vi "Every Value.vi"(8 "error in (no error)":errorcluster, 11 "prefix":string="DEV:") -> (0 "error out":errorcluster, 3 "values":map{string, refnum<class "NT Base.lvclass">}(c390))   [LabVIEW 2020]
uses:
  source/PV Data/NT Base/NT Base.lvclass
  source/PV Data/NT Scalar (Numeric)/NT Scalar (Numeric).lvclass
  C:/Users/eyw68381/source/repos/pvaccess-labview/labview/source/PV Data/NT Scalar/NT Scalar.lvclass
  C:/Users/eyw68381/source/repos/pvaccess-labview/labview/source/PV Data/NT Base/NT Base.lvclass
  source/PV Data/NT Scalar/NT Scalar.lvclass
  source/PV Data/NT Enum/NT Enum.lvclass
  source/PV Data/PV Data.lvlib
  source/PV Data/Value Fields.ctl
  source/PV Data/NT Scalar (Numeric)/Create - I64.vi
  source/PV Data/NT Scalar (Numeric)/Create - I32.vi
  source/PV Data/NT Scalar (Numeric)/Create - I16.vi
  source/PV Data/NT Scalar (Numeric)/Create - I8.vi
  source/PV Data/NT Scalar (Numeric)/Create - U16.vi
  source/PV Data/NT Scalar (Numeric)/Create - U8.vi
  source/PV Data/NT Scalar/Create - Boolean.vi
  source/PV Data/NT Scalar/Create - String.vi
  source/PV Data/NT Scalar (Numeric)/Create - DBL Array.vi
  source/PV Data/NT Scalar (Numeric)/Create - SGL Array.vi
  source/PV Data/NT Scalar (Numeric)/Create - I64 Array.vi
  source/PV Data/NT Scalar (Numeric)/Create - I32 Array.vi
  source/PV Data/NT Scalar (Numeric)/Create - I16 Array.vi
  source/PV Data/NT Scalar (Numeric)/Create - I8 Array.vi
  source/PV Data/NT Scalar (Numeric)/Create - U64 Array.vi
  source/PV Data/NT Scalar (Numeric)/Create - U32 Array.vi
  source/PV Data/NT Scalar (Numeric)/Create - U16 Array.vi
  source/PV Data/NT Scalar (Numeric)/Create - U8 Array.vi
  source/PV Data/NT Scalar/Create - Boolean Array.vi
  source/PV Data/NT Scalar/Create - String Array.vi
  source/PV Data/NT Enum/Create - Enum.vi
  source/PV Data/Display Form.ctl
  source/PV Data/NT Scalar (Numeric)/Create - SGL.vi
  source/PV Data/NT Scalar (Numeric)/Create - DBL.vi
  source/PV Data/NT Scalar (Numeric)/Create - U64.vi
  source/PV Data/NT Scalar (Numeric)/Create - U32.vi
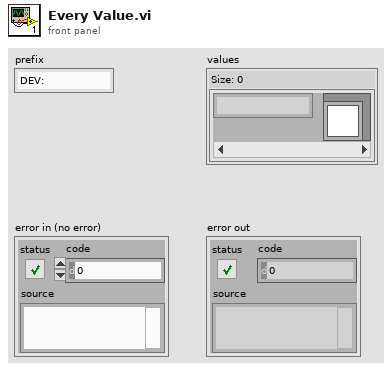
[diagram p1: front panel]
types:
  T1 = typedef "PV Access.lvlib/PV Data.lvlib/Display Form.ctl" = enum16{"Default", "String", "Binary", "Decimal", "Hex", "Exponential", "Engineering"}
  T2 = typedef "PV Access.lvlib/PV Data.lvlib/Value Fields.ctl" = cluster{"Display":bool, "Control":bool, "Alarm Limits":bool}
  T3 = typedef "PV Access.lvlib/PV Data.lvlib/Type Code.ctl" = enum8{"Null", "Bool", "BoolA", "Int8", "Int8A", "Int16", "Int16A", "Int32", "Int32A", "Int64", "Int64A", "UInt8", "UInt8A", "UInt16", "UInt16A", "UInt32", "UInt32A", "UInt64", "UInt64A", "Float32", "Float32A", "Float64", "Float64A", "String", "StringA", "Struct", "StructA", "Union", "UnionA", "Any", "AnyA"}
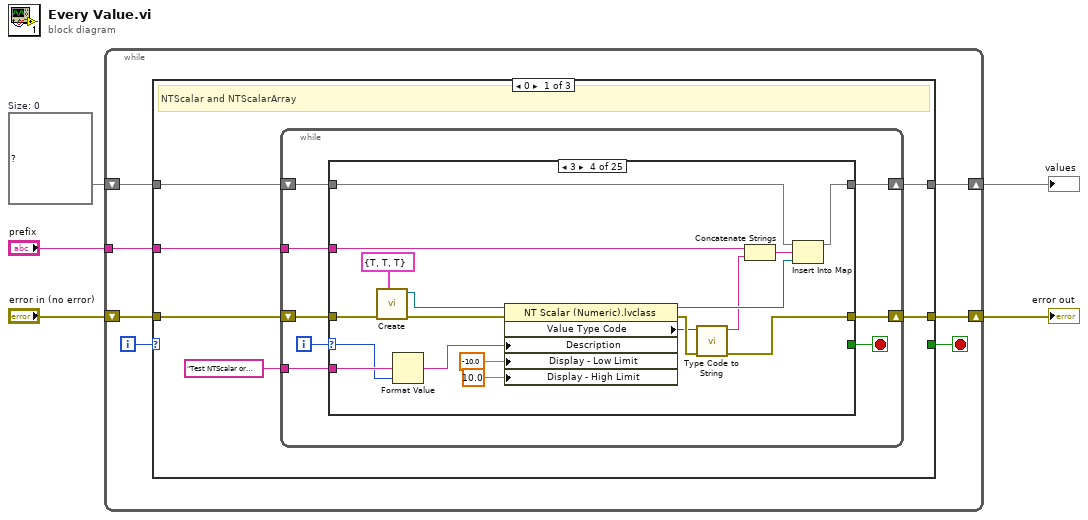
[diagram p0: block diagram]
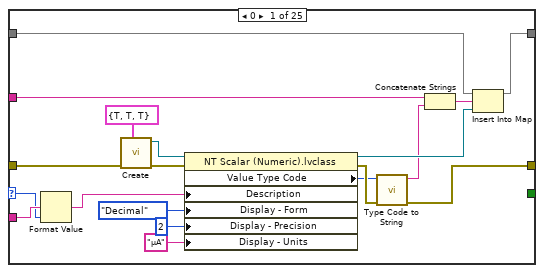
[diagram p2: hidden frame]
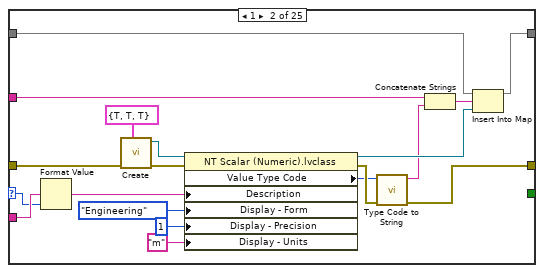
[diagram p3: hidden frame]
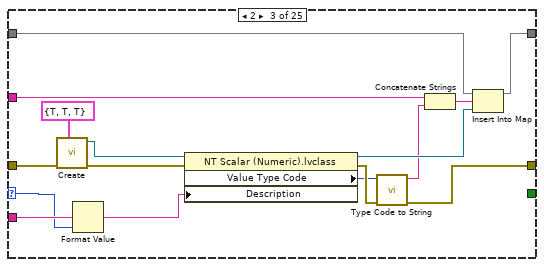
[diagram p4: hidden frame]
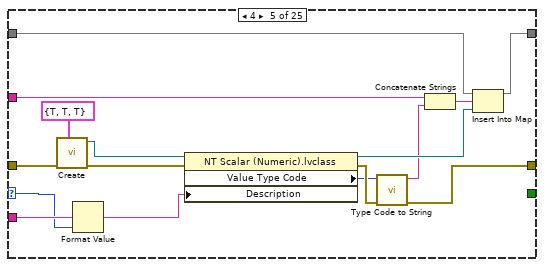
[diagram p5: hidden frame]
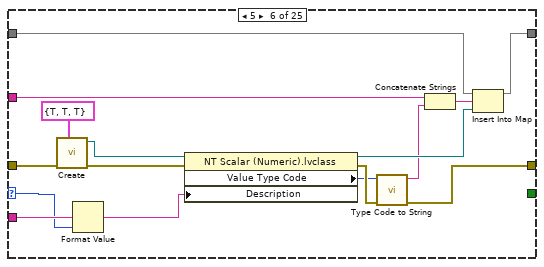
[diagram p6: hidden frame]
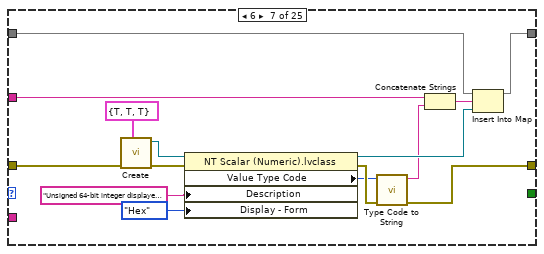
[diagram p7: hidden frame]
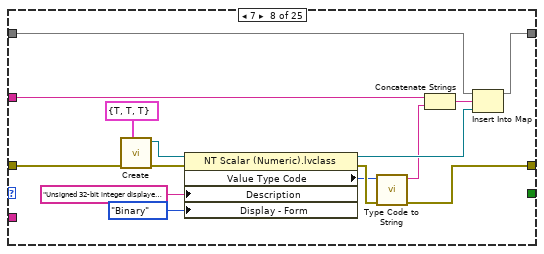
[diagram p8: hidden frame]
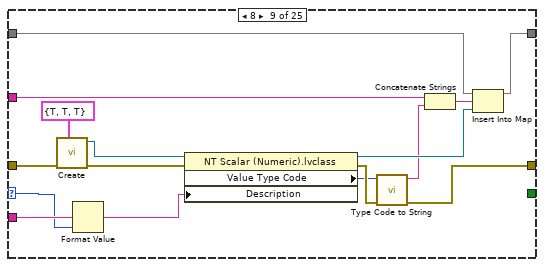
[diagram p9: hidden frame]
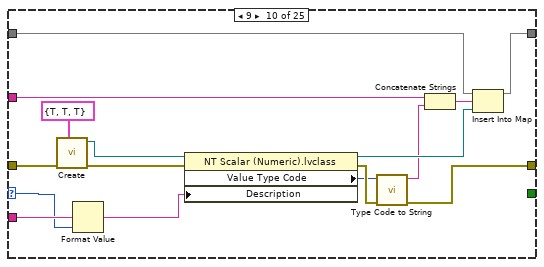
[diagram p10: hidden frame]
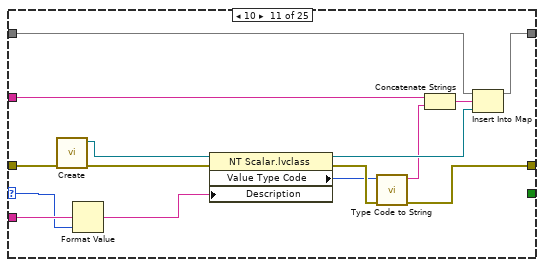
[diagram p11: hidden frame]
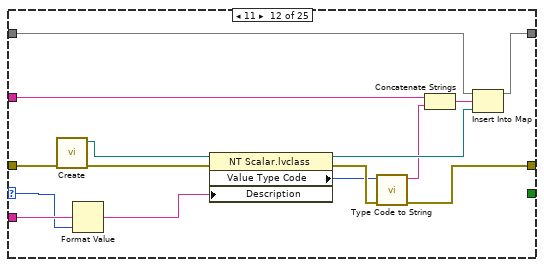
[diagram p12: hidden frame]
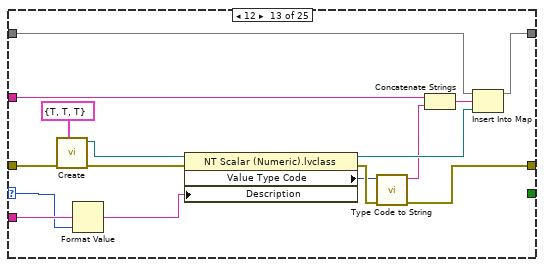
[diagram p13: hidden frame]
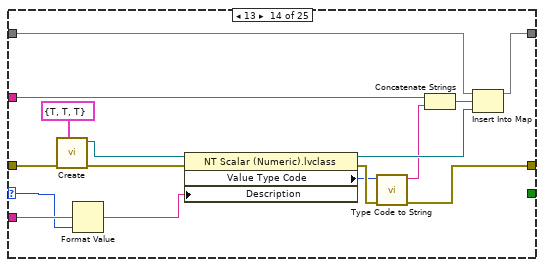
[diagram p14: hidden frame]
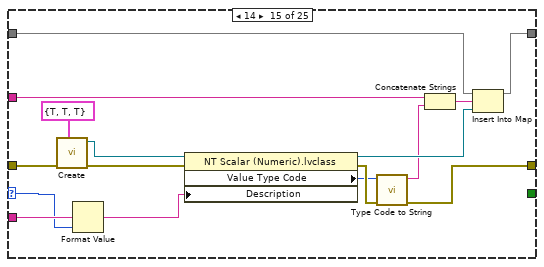
[diagram p15: hidden frame]
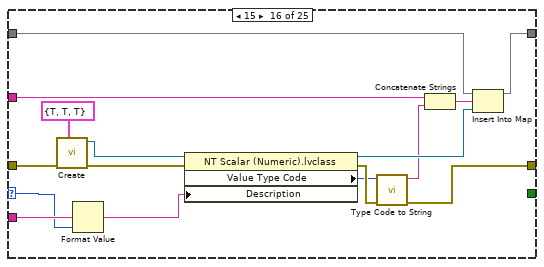
[diagram p16: hidden frame]
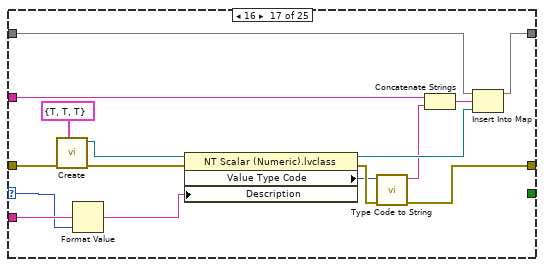
[diagram p17: hidden frame]
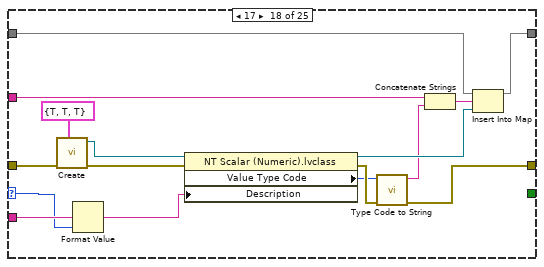
[diagram p18: hidden frame]
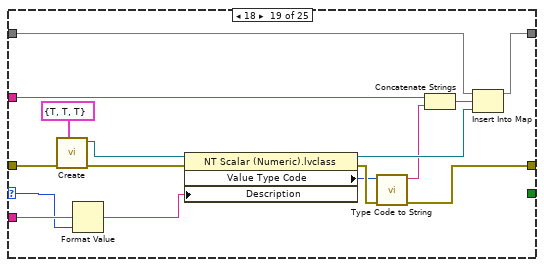
[diagram p19: hidden frame]
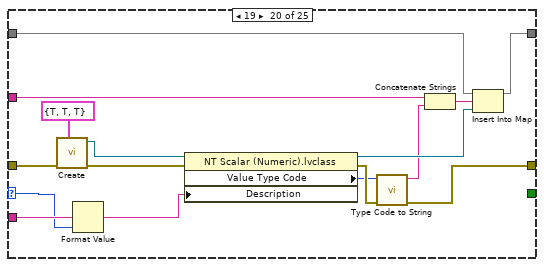
[diagram p20: hidden frame]
diagram:
  w3 = map{string, refnum<class "NT Base.lvclass">} {}  # Size: 0
  n1 = while {
    shift-right: [w11] -> w4
    shift-left: "error in (no error)" -> [w12]
    shift-right: [w9] -> w2
    shift-left: w3 -> [w10]
    tunnel: "prefix" -> [w6]
    i -> [w8]
    stop <- w7 stop-if-true
    n2 = case shown="0" w8 {
      tunnel: w12 -> [w18 w427 w430]
      tunnel: [w17 w420 w430] -> w11
      tunnel: w10 -> [w16 w426 w429]
      tunnel: [w15 w425 w429] -> w9
      tunnel: [_ _ TRUE] -> w7
      tunnel: w6 -> [w14 w424 _]
      frame 0 {
        # "NTScalar and NTScalarArray"
        n3 = while {
          shift-right: [w20] -> w17
          shift-left: w18 -> [w26]
          shift-right: [w21] -> w15
          shift-left: w16 -> [w22]
          tunnel: w14 -> [w23]
          tunnel: "Test NTScalar or NTScalarArray PV %d" ("Description") -> [w24]
          i -> [w25]
          stop <- w19 stop-if-true
          n4 = case shown="3" w25 {
            selector: w25 -> [w39 w58 w74 w92 w108 w124 _ _ w170 w186 w202 w217 w232 w248 w264 w280 w296 w312 w328 w344 w360 w376 w392 w407 _]
            tunnel: w26 -> [w45 w64 w80 w98 w114 w130 w145 w160 w176 w192 w207 w222 w238 w254 w270 w286 w302 w318 w334 w350 w366 w382 w397 w412 w415]
            tunnel: [w35 w54 w70 w88 w104 w120 w138 w153 w166 w182 w198 w213 w228 w244 w260 w276 w292 w308 w324 w340 w356 w372 w388 w403 w415] -> w20
            tunnel: w24 -> [w41 w60 w76 w94 w110 w126 _ _ w172 w188 w204 w219 w234 w250 w266 w282 w298 w314 w330 w346 w362 w378 w394 w409 _]
            tunnel: w23 -> [w37 w56 w72 w90 w106 w122 w140 w155 w168 w184 w200 w215 w230 w246 w262 w278 w294 w310 w326 w342 w358 w374 w390 w405 _]
            tunnel: w22 -> [w31 w50 w66 w84 w100 w116 w134 w149 w162 w178 w194 w209 w224 w240 w256 w272 w288 w304 w320 w336 w352 w368 w384 w399 w413]
            tunnel: [w30 w49 w65 w83 w99 w115 w133 w148 w161 w177 w193 w208 w223 w239 w255 w271 w287 w303 w319 w335 w351 w367 w383 w398 w413] -> w21
            tunnel: [_ _ _ _ _ _ _ _ _ _ _ _ _ _ _ _ _ _ _ _ _ _ _ _ TRUE] -> w19
            frame 0 {
              n5 = Format Value(format string=w41, value (0)=w39) -> (output string=w40:string)  [unwired: 1 in]
              n6 = call-poly "Create.vi"("fields"=T2 {"Display"=TRUE, "Control"=TRUE, "Alarm Limits"=TRUE}, "error in (no error)"=w45) -> ("error out"=w42:errorcluster, "NT Scalar (Numeric) out"=w43:refnum<class "NT Scalar (Numeric).lvclass">)  [unwired: 8 in]
              n7 = property class="NT Scalar (Numeric).lvclass"(reference=w43, error in=w42, "Description"=w40, "Display - Form"=Display_Form."Decimal" ("form"), "Display - Precision"=2 ("precision"), "Display - Units"="µA" ("units")) -> (reference out=w33:refnum<class "NT Scalar (Numeric).lvclass">, error out=w36:errorcluster, "Value Type Code"=w34:T3)
              n8 = call "Type Code to String.vi"("error in (no error)"=w36, "type code"=w34) -> ("error out"=w35:errorcluster, "string"=w32:string)  [unwired: 8 in]
              n9 = Concatenate Strings(w37, w32) -> (w38:string)
              n10 = Insert Into Map(map in=w31, key=w38, value=w33) -> (map out=w30:map{string, refnum<class "NT Base.lvclass">})  [unwired: 2 out]
            }
            frame 1 {
              n11 = Format Value(format string=w60, value (0)=w58) -> (output string=w59:string)  [unwired: 1 in]
              n12 = call-poly "Create.vi"("fields"=T2 {"Display"=TRUE, "Control"=TRUE, "Alarm Limits"=TRUE}, "error in (no error)"=w64) -> ("error out"=w61:errorcluster, "NT Scalar (Numeric) out"=w62:refnum<class "NT Scalar (Numeric).lvclass">)  [unwired: 8 in]
              n13 = property class="NT Scalar (Numeric).lvclass"(reference=w62, error in=w61, "Description"=w59, "Display - Form"=Display_Form."Engineering" ("form"), "Display - Precision"=1 ("precision"), "Display - Units"="m" ("units")) -> (reference out=w52:refnum<class "NT Scalar (Numeric).lvclass">, error out=w55:errorcluster, "Value Type Code"=w53:T3)
              n14 = call "Type Code to String.vi"("error in (no error)"=w55, "type code"=w53) -> ("error out"=w54:errorcluster, "string"=w51:string)  [unwired: 8 in]
              n15 = Concatenate Strings(w56, w51) -> (w57:string)
              n16 = Insert Into Map(map in=w50, key=w57, value=w52) -> (map out=w49:map{string, refnum<class "NT Base.lvclass">})  [unwired: 2 out]
            }
            frame 2 {
              n17 = call-poly "Create.vi"("fields"=T2 {"Display"=TRUE, "Control"=TRUE, "Alarm Limits"=TRUE}, "error in (no error)"=w80) -> ("error out"=w77:errorcluster, "NT Scalar (Numeric) out"=w78:refnum<class "NT Scalar (Numeric).lvclass">)  [unwired: 8 in]
              n18 = Format Value(format string=w76, value (0)=w74) -> (output string=w75:string)  [unwired: 1 in]
              n19 = property class="NT Scalar (Numeric).lvclass"(reference=w78, error in=w77, "Description"=w75) -> (reference out=w68:refnum<class "NT Scalar (Numeric).lvclass">, error out=w71:errorcluster, "Value Type Code"=w69:T3)
              n20 = call "Type Code to String.vi"("error in (no error)"=w71, "type code"=w69) -> ("error out"=w70:errorcluster, "string"=w67:string)  [unwired: 8 in]
              n21 = Concatenate Strings(w72, w67) -> (w73:string)
              n22 = Insert Into Map(map in=w66, key=w73, value=w68) -> (map out=w65:map{string, refnum<class "NT Base.lvclass">})  [unwired: 2 out]
            }
            frame 3 {
              n23 = call-poly "Create.vi"("fields"=T2 {"Display"=TRUE, "Control"=TRUE, "Alarm Limits"=TRUE}, "error in (no error)"=w98) -> ("error out"=w95:errorcluster, "NT Scalar (Numeric) out"=w96:refnum<class "NT Scalar (Numeric).lvclass">)  [unwired: 8 in]
              n24 = Format Value(format string=w94, value (0)=w92) -> (output string=w93:string)  [unwired: 1 in]
              n25 = property class="NT Scalar (Numeric).lvclass"(reference=w96, error in=w95, "Description"=w93, "Display - Low Limit"=-10.0 ("low limit"), "Display - High Limit"=10.0 ("high limit")) -> (reference out=w86:refnum<class "NT Scalar (Numeric).lvclass">, error out=w89:errorcluster, "Value Type Code"=w87:T3)
              n26 = call "Type Code to String.vi"("error in (no error)"=w89, "type code"=w87) -> ("error out"=w88:errorcluster, "string"=w85:string)  [unwired: 8 in]
              n27 = Concatenate Strings(w90, w85) -> (w91:string)
              n28 = Insert Into Map(map in=w84, key=w91, value=w86) -> (map out=w83:map{string, refnum<class "NT Base.lvclass">})  [unwired: 2 out]
            }
            frame 4 {
              n29 = call-poly "Create.vi"("fields"=T2 {"Display"=TRUE, "Control"=TRUE, "Alarm Limits"=TRUE}, "error in (no error)"=w114) -> ("error out"=w111:errorcluster, "NT Scalar (Numeric) out"=w112:refnum<class "NT Scalar (Numeric).lvclass">)  [unwired: 8 in]
              n30 = Format Value(format string=w110, value (0)=w108) -> (output string=w109:string)  [unwired: 1 in]
              n31 = property class="NT Scalar (Numeric).lvclass"(reference=w112, error in=w111, "Description"=w109) -> (reference out=w102:refnum<class "NT Scalar (Numeric).lvclass">, error out=w105:errorcluster, "Value Type Code"=w103:T3)
              n32 = call "Type Code to String.vi"("error in (no error)"=w105, "type code"=w103) -> ("error out"=w104:errorcluster, "string"=w101:string)  [unwired: 8 in]
              n33 = Concatenate Strings(w106, w101) -> (w107:string)
              n34 = Insert Into Map(map in=w100, key=w107, value=w102) -> (map out=w99:map{string, refnum<class "NT Base.lvclass">})  [unwired: 2 out]
            }
            frame 5 {
              n35 = call-poly "Create.vi"("fields"=T2 {"Display"=TRUE, "Control"=TRUE, "Alarm Limits"=TRUE}, "error in (no error)"=w130) -> ("error out"=w127:errorcluster, "NT Scalar (Numeric) out"=w128:refnum<class "NT Scalar (Numeric).lvclass">)  [unwired: 8 in]
              n36 = Format Value(format string=w126, value (0)=w124) -> (output string=w125:string)  [unwired: 1 in]
              n37 = property class="NT Scalar (Numeric).lvclass"(reference=w128, error in=w127, "Description"=w125) -> (reference out=w118:refnum<class "NT Scalar (Numeric).lvclass">, error out=w121:errorcluster, "Value Type Code"=w119:T3)
              n38 = call "Type Code to String.vi"("error in (no error)"=w121, "type code"=w119) -> ("error out"=w120:errorcluster, "string"=w117:string)  [unwired: 8 in]
              n39 = Concatenate Strings(w122, w117) -> (w123:string)
              n40 = Insert Into Map(map in=w116, key=w123, value=w118) -> (map out=w115:map{string, refnum<class "NT Base.lvclass">})  [unwired: 2 out]
            }
            frame 6 {
              n41 = call-poly "Create.vi"("fields"=T2 {"Display"=TRUE, "Control"=TRUE, "Alarm Limits"=TRUE}, "error in (no error)"=w145) -> ("error out"=w142:errorcluster, "NT Scalar (Numeric) out"=w143:refnum<class "NT Scalar (Numeric).lvclass">)  [unwired: 8 in]
              n42 = property class="NT Scalar (Numeric).lvclass"(reference=w143, error in=w142, "Description"="Unsigned 64-bit integer displayed in hexadecimal" ("description"), "Display - Form"=Display_Form."Hex" ("form")) -> (reference out=w136:refnum<class "NT Scalar (Numeric).lvclass">, error out=w139:errorcluster, "Value Type Code"=w137:T3)
              n43 = call "Type Code to String.vi"("error in (no error)"=w139, "type code"=w137) -> ("error out"=w138:errorcluster, "string"=w135:string)  [unwired: 8 in]
              n44 = Concatenate Strings(w140, w135) -> (w141:string)
              n45 = Insert Into Map(map in=w134, key=w141, value=w136) -> (map out=w133:map{string, refnum<class "NT Base.lvclass">})  [unwired: 2 out]
            }
            frame 7 {
              n46 = call-poly "Create.vi"("fields"=T2 {"Display"=TRUE, "Control"=TRUE, "Alarm Limits"=TRUE}, "error in (no error)"=w160) -> ("error out"=w157:errorcluster, "NT Scalar (Numeric) out"=w158:refnum<class "NT Scalar (Numeric).lvclass">)  [unwired: 8 in]
              n47 = property class="NT Scalar (Numeric).lvclass"(reference=w158, error in=w157, "Description"="Unsigned 32-bit integer displayed in binary" ("description"), "Display - Form"=Display_Form."Binary" ("form")) -> (reference out=w151:refnum<class "NT Scalar (Numeric).lvclass">, error out=w154:errorcluster, "Value Type Code"=w152:T3)
              n48 = call "Type Code to String.vi"("error in (no error)"=w154, "type code"=w152) -> ("error out"=w153:errorcluster, "string"=w150:string)  [unwired: 8 in]
              n49 = Concatenate Strings(w155, w150) -> (w156:string)
              n50 = Insert Into Map(map in=w149, key=w156, value=w151) -> (map out=w148:map{string, refnum<class "NT Base.lvclass">})  [unwired: 2 out]
            }
            frame 8 {
              n51 = call-poly "Create.vi"("fields"=T2 {"Display"=TRUE, "Control"=TRUE, "Alarm Limits"=TRUE}, "error in (no error)"=w176) -> ("error out"=w173:errorcluster, "NT Scalar (Numeric) out"=w174:refnum<class "NT Scalar (Numeric).lvclass">)  [unwired: 8 in]
              n52 = Format Value(format string=w172, value (0)=w170) -> (output string=w171:string)  [unwired: 1 in]
              n53 = property class="NT Scalar (Numeric).lvclass"(reference=w174, error in=w173, "Description"=w171) -> (reference out=w164:refnum<class "NT Scalar (Numeric).lvclass">, error out=w167:errorcluster, "Value Type Code"=w165:T3)
              n54 = call "Type Code to String.vi"("error in (no error)"=w167, "type code"=w165) -> ("error out"=w166:errorcluster, "string"=w163:string)  [unwired: 8 in]
              n55 = Concatenate Strings(w168, w163) -> (w169:string)
              n56 = Insert Into Map(map in=w162, key=w169, value=w164) -> (map out=w161:map{string, refnum<class "NT Base.lvclass">})  [unwired: 2 out]
            }
            frame 9 {
              n57 = call-poly "Create.vi"("fields"=T2 {"Display"=TRUE, "Control"=TRUE, "Alarm Limits"=TRUE}, "error in (no error)"=w192) -> ("error out"=w189:errorcluster, "NT Scalar (Numeric) out"=w190:refnum<class "NT Scalar (Numeric).lvclass">)  [unwired: 8 in]
              n58 = Format Value(format string=w188, value (0)=w186) -> (output string=w187:string)  [unwired: 1 in]
              n59 = property class="NT Scalar (Numeric).lvclass"(reference=w190, error in=w189, "Description"=w187) -> (reference out=w180:refnum<class "NT Scalar (Numeric).lvclass">, error out=w183:errorcluster, "Value Type Code"=w181:T3)
              n60 = call "Type Code to String.vi"("error in (no error)"=w183, "type code"=w181) -> ("error out"=w182:errorcluster, "string"=w179:string)  [unwired: 8 in]
              n61 = Concatenate Strings(w184, w179) -> (w185:string)
              n62 = Insert Into Map(map in=w178, key=w185, value=w180) -> (map out=w177:map{string, refnum<class "NT Base.lvclass">})  [unwired: 2 out]
            }
            frame 10 {
              n63 = call-poly "Create.vi"("error in (no error)"=w207) -> ("error out"=w205:errorcluster, "NT Scalar out"=w206:refnum<class "NT Scalar.lvclass">)  [unwired: 9 in]
              n64 = Format Value(format string=w204, value (0)=w202) -> (output string=w203:string)  [unwired: 1 in]
              n65 = property class="NT Scalar.lvclass"(reference=w206, error in=w205, "Description"=w203) -> (reference out=w196:refnum<class "NT Scalar.lvclass">, error out=w199:errorcluster, "Value Type Code"=w197:T3)
              n66 = call "Type Code to String.vi"("error in (no error)"=w199, "type code"=w197) -> ("error out"=w198:errorcluster, "string"=w195:string)  [unwired: 8 in]
              n67 = Concatenate Strings(w200, w195) -> (w201:string)
              n68 = Insert Into Map(map in=w194, key=w201, value=w196) -> (map out=w193:map{string, refnum<class "NT Base.lvclass">})  [unwired: 2 out]
            }
            frame 11 {
              n69 = call-poly "Create.vi"("error in (no error)"=w222) -> ("error out"=w220:errorcluster, "NT Scalar out"=w221:refnum<class "NT Scalar.lvclass">)  [unwired: 9 in]
              n70 = Format Value(format string=w219, value (0)=w217) -> (output string=w218:string)  [unwired: 1 in]
              n71 = property class="NT Scalar.lvclass"(reference=w221, error in=w220, "Description"=w218) -> (reference out=w211:refnum<class "NT Scalar.lvclass">, error out=w214:errorcluster, "Value Type Code"=w212:T3)
              n72 = call "Type Code to String.vi"("error in (no error)"=w214, "type code"=w212) -> ("error out"=w213:errorcluster, "string"=w210:string)  [unwired: 8 in]
              n73 = Concatenate Strings(w215, w210) -> (w216:string)
              n74 = Insert Into Map(map in=w209, key=w216, value=w211) -> (map out=w208:map{string, refnum<class "NT Base.lvclass">})  [unwired: 2 out]
            }
            frame 12 {
              n75 = call-poly "Create.vi"("fields"=T2 {"Display"=TRUE, "Control"=TRUE, "Alarm Limits"=TRUE}, "error in (no error)"=w238) -> ("error out"=w235:errorcluster, "NT Scalar (Numeric) out"=w236:refnum<class "NT Scalar (Numeric).lvclass">)  [unwired: 8 in]
              n76 = Format Value(format string=w234, value (0)=w232) -> (output string=w233:string)  [unwired: 1 in]
              n77 = property class="NT Scalar (Numeric).lvclass"(reference=w236, error in=w235, "Description"=w233) -> (reference out=w226:refnum<class "NT Scalar (Numeric).lvclass">, error out=w229:errorcluster, "Value Type Code"=w227:T3)
              n78 = call "Type Code to String.vi"("error in (no error)"=w229, "type code"=w227) -> ("error out"=w228:errorcluster, "string"=w225:string)  [unwired: 8 in]
              n79 = Concatenate Strings(w230, w225) -> (w231:string)
              n80 = Insert Into Map(map in=w224, key=w231, value=w226) -> (map out=w223:map{string, refnum<class "NT Base.lvclass">})  [unwired: 2 out]
            }
            frame 13 {
              n81 = call-poly "Create.vi"("fields"=T2 {"Display"=TRUE, "Control"=TRUE, "Alarm Limits"=TRUE}, "error in (no error)"=w254) -> ("error out"=w251:errorcluster, "NT Scalar (Numeric) out"=w252:refnum<class "NT Scalar (Numeric).lvclass">)  [unwired: 8 in]
              n82 = Format Value(format string=w250, value (0)=w248) -> (output string=w249:string)  [unwired: 1 in]
              n83 = property class="NT Scalar (Numeric).lvclass"(reference=w252, error in=w251, "Description"=w249) -> (reference out=w242:refnum<class "NT Scalar (Numeric).lvclass">, error out=w245:errorcluster, "Value Type Code"=w243:T3)
              n84 = call "Type Code to String.vi"("error in (no error)"=w245, "type code"=w243) -> ("error out"=w244:errorcluster, "string"=w241:string)  [unwired: 8 in]
              n85 = Concatenate Strings(w246, w241) -> (w247:string)
              n86 = Insert Into Map(map in=w240, key=w247, value=w242) -> (map out=w239:map{string, refnum<class "NT Base.lvclass">})  [unwired: 2 out]
            }
            frame 14 {
              n87 = call-poly "Create.vi"("fields"=T2 {"Display"=TRUE, "Control"=TRUE, "Alarm Limits"=TRUE}, "error in (no error)"=w270) -> ("error out"=w267:errorcluster, "NT Scalar (Numeric) out"=w268:refnum<class "NT Scalar (Numeric).lvclass">)  [unwired: 8 in]
              n88 = Format Value(format string=w266, value (0)=w264) -> (output string=w265:string)  [unwired: 1 in]
              n89 = property class="NT Scalar (Numeric).lvclass"(reference=w268, error in=w267, "Description"=w265) -> (reference out=w258:refnum<class "NT Scalar (Numeric).lvclass">, error out=w261:errorcluster, "Value Type Code"=w259:T3)
              n90 = call "Type Code to String.vi"("error in (no error)"=w261, "type code"=w259) -> ("error out"=w260:errorcluster, "string"=w257:string)  [unwired: 8 in]
              n91 = Concatenate Strings(w262, w257) -> (w263:string)
              n92 = Insert Into Map(map in=w256, key=w263, value=w258) -> (map out=w255:map{string, refnum<class "NT Base.lvclass">})  [unwired: 2 out]
            }
            frame 15 {
              n93 = call-poly "Create.vi"("fields"=T2 {"Display"=TRUE, "Control"=TRUE, "Alarm Limits"=TRUE}, "error in (no error)"=w286) -> ("error out"=w283:errorcluster, "NT Scalar (Numeric) out"=w284:refnum<class "NT Scalar (Numeric).lvclass">)  [unwired: 8 in]
              n94 = Format Value(format string=w282, value (0)=w280) -> (output string=w281:string)  [unwired: 1 in]
              n95 = property class="NT Scalar (Numeric).lvclass"(reference=w284, error in=w283, "Description"=w281) -> (reference out=w274:refnum<class "NT Scalar (Numeric).lvclass">, error out=w277:errorcluster, "Value Type Code"=w275:T3)
              n96 = call "Type Code to String.vi"("error in (no error)"=w277, "type code"=w275) -> ("error out"=w276:errorcluster, "string"=w273:string)  [unwired: 8 in]
              n97 = Concatenate Strings(w278, w273) -> (w279:string)
              n98 = Insert Into Map(map in=w272, key=w279, value=w274) -> (map out=w271:map{string, refnum<class "NT Base.lvclass">})  [unwired: 2 out]
            }
            frame 16 {
              n99 = call-poly "Create.vi"("fields"=T2 {"Display"=TRUE, "Control"=TRUE, "Alarm Limits"=TRUE}, "error in (no error)"=w302) -> ("error out"=w299:errorcluster, "NT Scalar (Numeric) out"=w300:refnum<class "NT Scalar (Numeric).lvclass">)  [unwired: 8 in]
              n100 = Format Value(format string=w298, value (0)=w296) -> (output string=w297:string)  [unwired: 1 in]
              n101 = property class="NT Scalar (Numeric).lvclass"(reference=w300, error in=w299, "Description"=w297) -> (reference out=w290:refnum<class "NT Scalar (Numeric).lvclass">, error out=w293:errorcluster, "Value Type Code"=w291:T3)
              n102 = call "Type Code to String.vi"("error in (no error)"=w293, "type code"=w291) -> ("error out"=w292:errorcluster, "string"=w289:string)  [unwired: 8 in]
              n103 = Concatenate Strings(w294, w289) -> (w295:string)
              n104 = Insert Into Map(map in=w288, key=w295, value=w290) -> (map out=w287:map{string, refnum<class "NT Base.lvclass">})  [unwired: 2 out]
            }
            frame 17 {
              n105 = call-poly "Create.vi"("fields"=T2 {"Display"=TRUE, "Control"=TRUE, "Alarm Limits"=TRUE}, "error in (no error)"=w318) -> ("error out"=w315:errorcluster, "NT Scalar (Numeric) out"=w316:refnum<class "NT Scalar (Numeric).lvclass">)  [unwired: 8 in]
              n106 = Format Value(format string=w314, value (0)=w312) -> (output string=w313:string)  [unwired: 1 in]
              n107 = property class="NT Scalar (Numeric).lvclass"(reference=w316, error in=w315, "Description"=w313) -> (reference out=w306:refnum<class "NT Scalar (Numeric).lvclass">, error out=w309:errorcluster, "Value Type Code"=w307:T3)
              n108 = call "Type Code to String.vi"("error in (no error)"=w309, "type code"=w307) -> ("error out"=w308:errorcluster, "string"=w305:string)  [unwired: 8 in]
              n109 = Concatenate Strings(w310, w305) -> (w311:string)
              n110 = Insert Into Map(map in=w304, key=w311, value=w306) -> (map out=w303:map{string, refnum<class "NT Base.lvclass">})  [unwired: 2 out]
            }
            frame 18 {
              n111 = call-poly "Create.vi"("fields"=T2 {"Display"=TRUE, "Control"=TRUE, "Alarm Limits"=TRUE}, "error in (no error)"=w334) -> ("error out"=w331:errorcluster, "NT Scalar (Numeric) out"=w332:refnum<class "NT Scalar (Numeric).lvclass">)  [unwired: 8 in]
              n112 = Format Value(format string=w330, value (0)=w328) -> (output string=w329:string)  [unwired: 1 in]
              n113 = property class="NT Scalar (Numeric).lvclass"(reference=w332, error in=w331, "Description"=w329) -> (reference out=w322:refnum<class "NT Scalar (Numeric).lvclass">, error out=w325:errorcluster, "Value Type Code"=w323:T3)
              n114 = call "Type Code to String.vi"("error in (no error)"=w325, "type code"=w323) -> ("error out"=w324:errorcluster, "string"=w321:string)  [unwired: 8 in]
              n115 = Concatenate Strings(w326, w321) -> (w327:string)
              n116 = Insert Into Map(map in=w320, key=w327, value=w322) -> (map out=w319:map{string, refnum<class "NT Base.lvclass">})  [unwired: 2 out]
            }
            frame 19 {
              n117 = call-poly "Create.vi"("fields"=T2 {"Display"=TRUE, "Control"=TRUE, "Alarm Limits"=TRUE}, "error in (no error)"=w350) -> ("error out"=w347:errorcluster, "NT Scalar (Numeric) out"=w348:refnum<class "NT Scalar (Numeric).lvclass">)  [unwired: 8 in]
              n118 = Format Value(format string=w346, value (0)=w344) -> (output string=w345:string)  [unwired: 1 in]
              n119 = property class="NT Scalar (Numeric).lvclass"(reference=w348, error in=w347, "Description"=w345) -> (reference out=w338:refnum<class "NT Scalar (Numeric).lvclass">, error out=w341:errorcluster, "Value Type Code"=w339:T3)
              n120 = call "Type Code to String.vi"("error in (no error)"=w341, "type code"=w339) -> ("error out"=w340:errorcluster, "string"=w337:string)  [unwired: 8 in]
              n121 = Concatenate Strings(w342, w337) -> (w343:string)
              n122 = Insert Into Map(map in=w336, key=w343, value=w338) -> (map out=w335:map{string, refnum<class "NT Base.lvclass">})  [unwired: 2 out]
            }
            frame 20 {
              n123 = call-poly "Create.vi"("fields"=T2 {"Display"=TRUE, "Control"=TRUE, "Alarm Limits"=TRUE}, "error in (no error)"=w366) -> ("error out"=w363:errorcluster, "NT Scalar (Numeric) out"=w364:refnum<class "NT Scalar (Numeric).lvclass">)  [unwired: 8 in]
              n124 = Format Value(format string=w362, value (0)=w360) -> (output string=w361:string)  [unwired: 1 in]
              n125 = property class="NT Scalar (Numeric).lvclass"(reference=w364, error in=w363, "Description"=w361) -> (reference out=w354:refnum<class "NT Scalar (Numeric).lvclass">, error out=w357:errorcluster, "Value Type Code"=w355:T3)
              n126 = call "Type Code to String.vi"("error in (no error)"=w357, "type code"=w355) -> ("error out"=w356:errorcluster, "string"=w353:string)  [unwired: 8 in]
              n127 = Concatenate Strings(w358, w353) -> (w359:string)
              n128 = Insert Into Map(map in=w352, key=w359, value=w354) -> (map out=w351:map{string, refnum<class "NT Base.lvclass">})  [unwired: 2 out]
            }
            frame 21 {
              n129 = call-poly "Create.vi"("fields"=T2 {"Display"=TRUE, "Control"=TRUE, "Alarm Limits"=TRUE}, "error in (no error)"=w382) -> ("error out"=w379:errorcluster, "NT Scalar (Numeric) out"=w380:refnum<class "NT Scalar (Numeric).lvclass">)  [unwired: 8 in]
              n130 = Format Value(format string=w378, value (0)=w376) -> (output string=w377:string)  [unwired: 1 in]
              n131 = property class="NT Scalar (Numeric).lvclass"(reference=w380, error in=w379, "Description"=w377) -> (reference out=w370:refnum<class "NT Scalar (Numeric).lvclass">, error out=w373:errorcluster, "Value Type Code"=w371:T3)
              n132 = call "Type Code to String.vi"("error in (no error)"=w373, "type code"=w371) -> ("error out"=w372:errorcluster, "string"=w369:string)  [unwired: 8 in]
              n133 = Concatenate Strings(w374, w369) -> (w375:string)
              n134 = Insert Into Map(map in=w368, key=w375, value=w370) -> (map out=w367:map{string, refnum<class "NT Base.lvclass">})  [unwired: 2 out]
            }
            frame 22 {
              n135 = call-poly "Create.vi"("error in (no error)"=w397) -> ("error out"=w395:errorcluster, "NT Scalar out"=w396:refnum<class "NT Scalar.lvclass">)  [unwired: 9 in]
              n136 = Format Value(format string=w394, value (0)=w392) -> (output string=w393:string)  [unwired: 1 in]
              n137 = property class="NT Scalar.lvclass"(reference=w396, error in=w395, "Description"=w393) -> (reference out=w386:refnum<class "NT Scalar.lvclass">, error out=w389:errorcluster, "Value Type Code"=w387:T3)
              n138 = call "Type Code to String.vi"("error in (no error)"=w389, "type code"=w387) -> ("error out"=w388:errorcluster, "string"=w385:string)  [unwired: 8 in]
              n139 = Concatenate Strings(w390, w385) -> (w391:string)
              n140 = Insert Into Map(map in=w384, key=w391, value=w386) -> (map out=w383:map{string, refnum<class "NT Base.lvclass">})  [unwired: 2 out]
            }
            frame 23 {
              n141 = call-poly "Create.vi"("error in (no error)"=w412) -> ("error out"=w410:errorcluster, "NT Scalar out"=w411:refnum<class "NT Scalar.lvclass">)  [unwired: 9 in]
              n142 = Format Value(format string=w409, value (0)=w407) -> (output string=w408:string)  [unwired: 1 in]
              n143 = property class="NT Scalar.lvclass"(reference=w411, error in=w410, "Description"=w408) -> (reference out=w401:refnum<class "NT Scalar.lvclass">, error out=w404:errorcluster, "Value Type Code"=w402:T3)
              n144 = call "Type Code to String.vi"("error in (no error)"=w404, "type code"=w402) -> ("error out"=w403:errorcluster, "string"=w400:string)  [unwired: 8 in]
              n145 = Concatenate Strings(w405, w400) -> (w406:string)
              n146 = Insert Into Map(map in=w399, key=w406, value=w401) -> (map out=w398:map{string, refnum<class "NT Base.lvclass">})  [unwired: 2 out]
            }
            frame Default {
            }
          }
        }
      }
      frame 1 {
        # "NT Enum"
        n147 = call-poly "Create.vi"("error in (no error)"=w427, "choices"=string[] ["A", "B", "C"]) -> ("error out"=w422:errorcluster, "NT Enum out"=w423:refnum<class "NT Enum.lvclass">)  [unwired: 8 in]
        n148 = property class="NT Enum.lvclass"(reference=w423, error in=w422, "Description"="Test NTEnum") -> (reference out=w419:refnum<class "NT Enum.lvclass">, error out=w420:errorcluster)
        n149 = Concatenate Strings(w424, "ENUM" ("string")) -> (w421:string)
        n150 = Insert Into Map(map in=w426, key=w421, value=w419) -> (map out=w425:map{string, refnum<class "NT Base.lvclass">})  [unwired: 2 out]
      }
      frame Default {
      }
    }
  }
  "error out" <- w4
  "values" <- w2
